vi "lab3.vi"() -> ()   [LabVIEW 2026]
uses:
  <vilib>/express/express analysis/Spectral/Block/exnSpectralBlock spectral measurements power poly.vi
  <vilib>/express/express analysis/Spectral/XNode/ExpressSpectralMeasurementsBlockNode.xnode
  <vilib>/express/express analysis/Spectral/Block/exnSpectralBlock spectral measurements power DDT.vi
panel:
  out "Filtered Signal 2":dynamicdata(graph) caption="Filtered Signal"
  out "Waveform Graph":dynamicdata(graph)
  out "Filtered Signal":dynamicdata(graph)
  out "data":dynamicdata(graph)
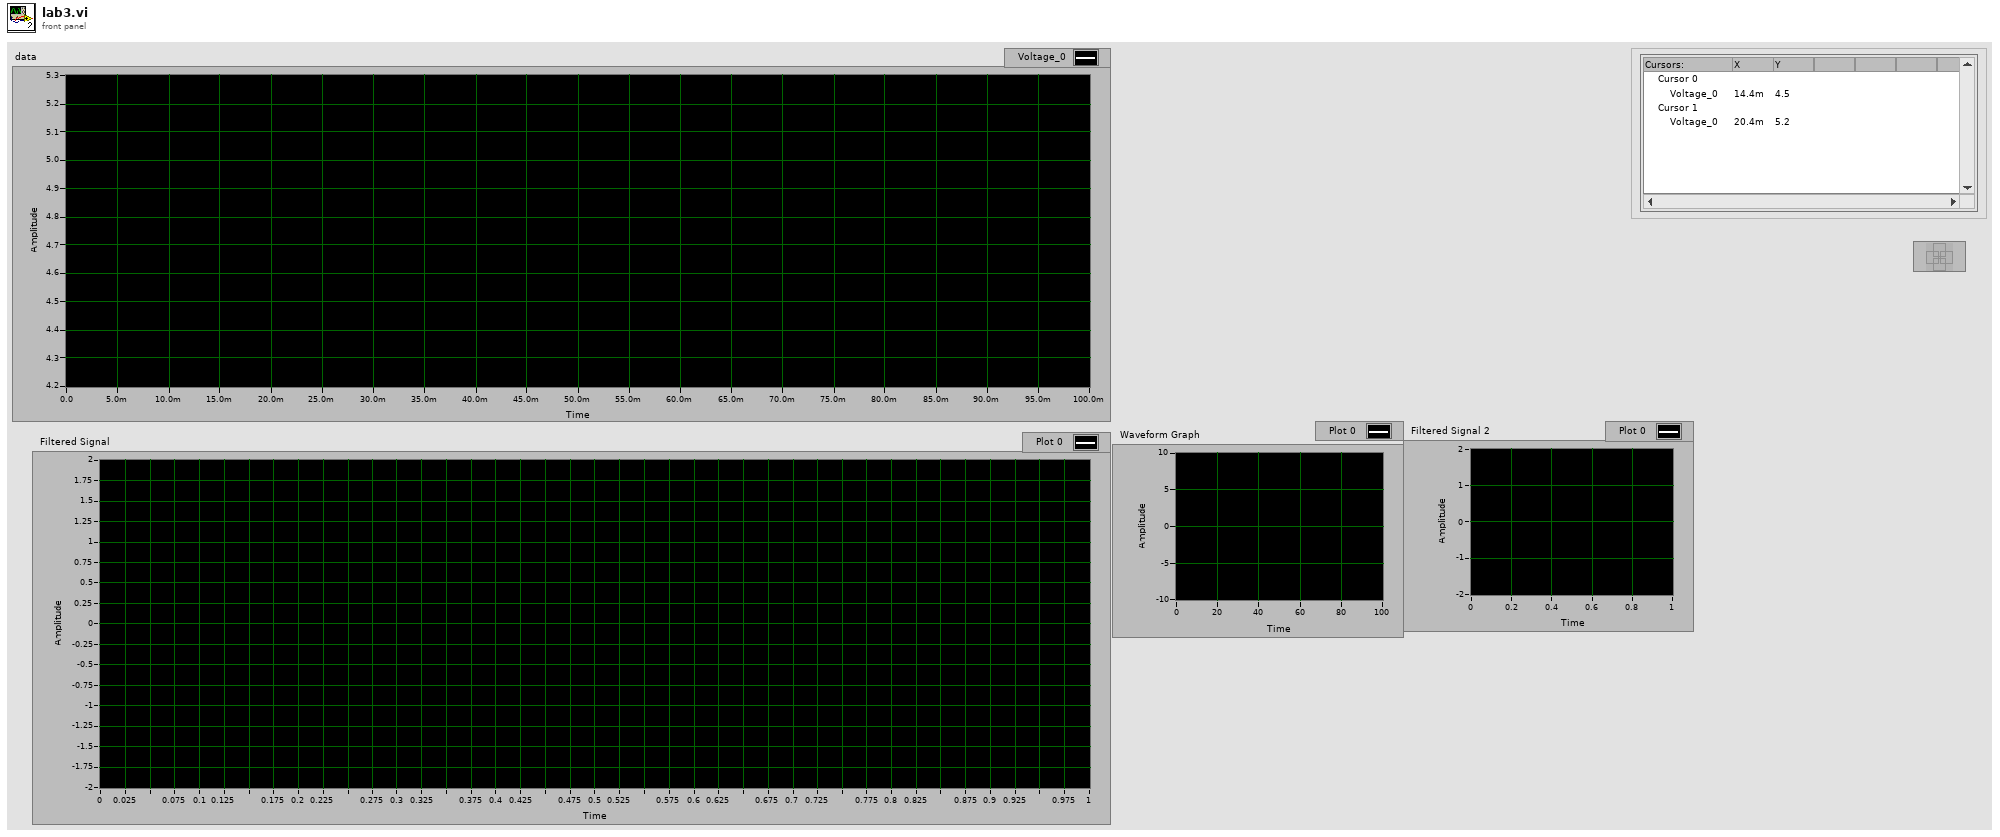
[diagram p1: front panel]
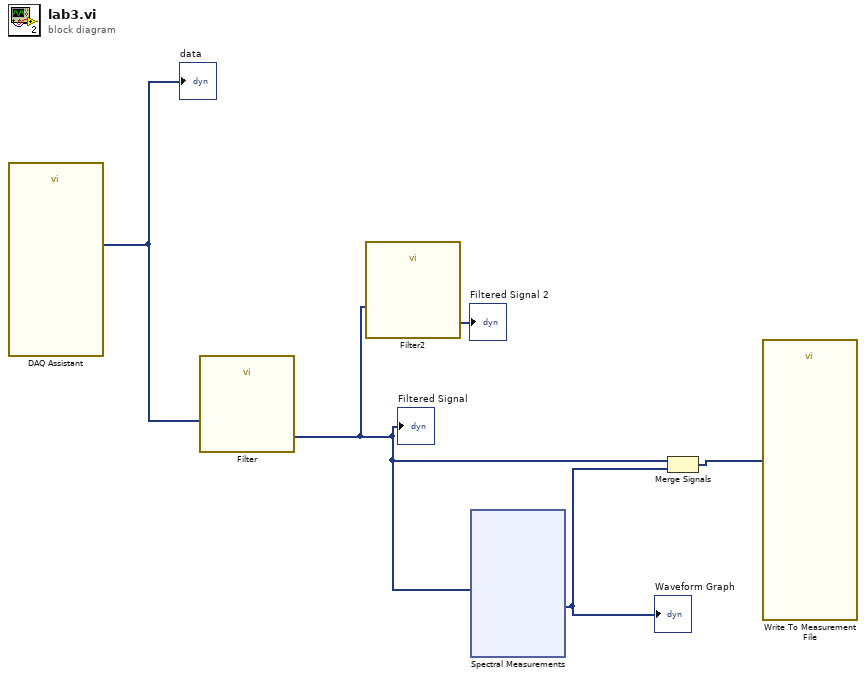
[diagram p0: block diagram]
diagram:
  n1 = call "DAQ Assistant"() -> ("data"=w5:dynamicdata)  [unwired: 17 in, 2 out]
  "data" <- w5
  n2 = call "Filter"("Signal"=w5) -> ("Filtered Signal"=w2:dynamicdata)  [unwired: 9 in, 1 out]
  "Filtered Signal" <- w2
  n3 = call "Filter2"("Signal"=w2) -> ("Filtered Signal"=→"Filtered Signal 2":dynamicdata)  [unwired: 9 in, 1 out]
  n4 = xnode "Spectral Measurements"("Signals"=w2) -> ("Power Spectrum"=w3:dynamicdata)  [unwired: 1 in, 1 out]
  "Waveform Graph" <- w3
  n5 = Merge Signals(w2, w3) -> (w4:dynamicdata)
  n6 = call "Write To Measurement File"("Signals"=w4) -> ()  [unwired: 16 in, 3 out]
